vi "set Marker Frequency Count.vi"(6 "On?":bool, 8 "error in (no error)":errorcluster, 10 "Index":i32, 11 "FSV-40N in":refnum<class "FSV-40N.lvclass">) -> (0 "error out":errorcluster, 3 "FSV-40N out":refnum<class "FSV-40N.lvclass">)   [LabVIEW 2023, in "Spectrum Analyzer.lvlib" / "FSV-40N.lvclass"]
uses:
  FSV-40N.lvclass
  FSV-40N.lvclass/FSV-40N.ctl
  <vilib>/ErrorRing/Error Ring.xnode
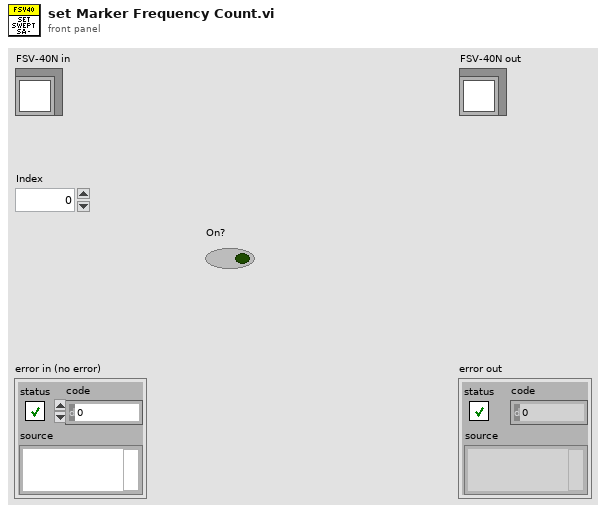
[diagram p1: front panel]
types:
  T1 = typedef "Spectrum Analyzer.lvlib/TYPE Marker Type Map.ctl" = map{i32, T2}
  T2 = typedef "Spectrum Analyzer.lvlib/TYPE Marker Control Mode.ctl" = enum16{"Normal", "Delta", "Off"}
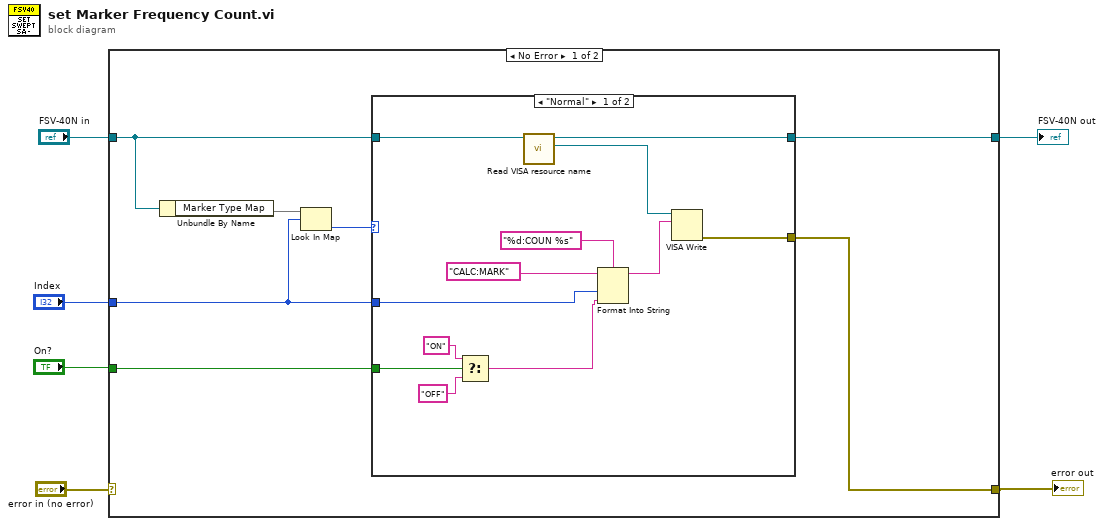
[diagram p0: block diagram]
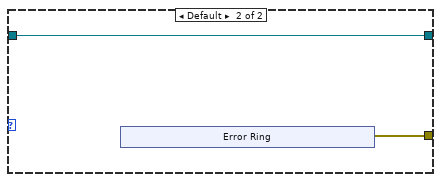
[diagram p2: hidden frame]
diagram:
  n1 = case shown="No Error" "error in (no error)" {
    selector: "error in (no error)" -> [_ w29]
    tunnel: "FSV-40N in" -> [w10 w30]
    tunnel: [w12 w30] -> w5
    tunnel: [w13 w29] -> w3
    tunnel: "On?" -> [w11 _]
    tunnel: "Index" -> [w7 _]
    frame No Error {
      n2 = Unbundle By Name(w10) -> ("Marker Type Map"=w9:T1)
      n3 = Look In Map(map=w9, key=w7) -> (value=w8:T2)  [unwired: 1 in, 1 out]
      n4 = case shown="\"Normal\"" w8 {
        tunnel: [w23 w26] -> w13
        tunnel: [w21 w27] -> w12
        tunnel: w11 -> [w19 _]
        tunnel: w10 -> [w16 w27]
        tunnel: w7 -> [w15 _]
        frame "Normal" {
          n5 = Select(t="ON" ("initial string"), s=w19, f="OFF" ("initial string")) -> (s? t:f=w14:string)
          n6 = call "Read VISA resource name.vi"("FSV-40N in"=w16) -> ("VISA resource name"=w22:refnum<visa-resource-name>, "FSV-40N out"=w21:refnum<class "FSV-40N.lvclass">)  [unwired: 8 in, 1 out]
          n7 = Format Into String(format string="%d:COUN %s", initial string="CALC:MARK", w15, w14) -> (resulting string=w24:string)  [unwired: 1 in, 1 out]
          n8 = VISA Write(VISA resource name=w22, write buffer=w24) -> (error out=w23:errorcluster)  [unwired: 1 in, 2 out]
        }
        frame Default {
          n9 = xnode "Error Ring"() -> ("error out"=w26:errorcluster)
        }
      }
    }
    frame Error {
    }
  }
  "error out" <- w3
  "FSV-40N out" <- w5
